vi "XMLPublishNode.vi"(8 "Error In":errorcluster, 9 "parent opcua path":string, 10 "OPC UA server refnum in":refnum<k21>, 11 "DOM node":refnum<k20>) -> (0 "Error Out":errorcluster, 2 "OPC UA server refnum out":refnum<k21>, 3 "DOM node (dup)":refnum<k20>)   [LabVIEW 2014, in "OPCUA XML(dev).lvlib"]
uses:
  OPCUA XML(dev).lvlib
  <resource>/objmgr/DOMUserDefRef.rc
  <vilib>/xml/NI_XML.lvlib
  <vilib>/xml/Close Reference(Node).vi
  <vilib>/OPCUA/NI OPC UA Server.lvlib
  <vilib>/xml/Close Reference(NNMap).vi
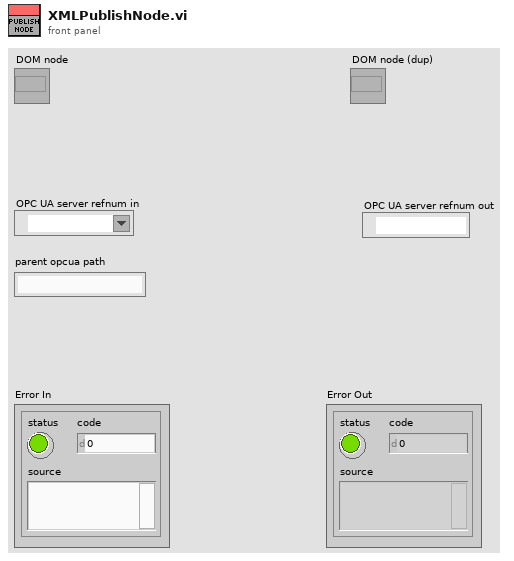
[diagram p1: front panel]
types:
  T1 = cluster{"name":string, "data type":u16, "access level":u16, "description":string}
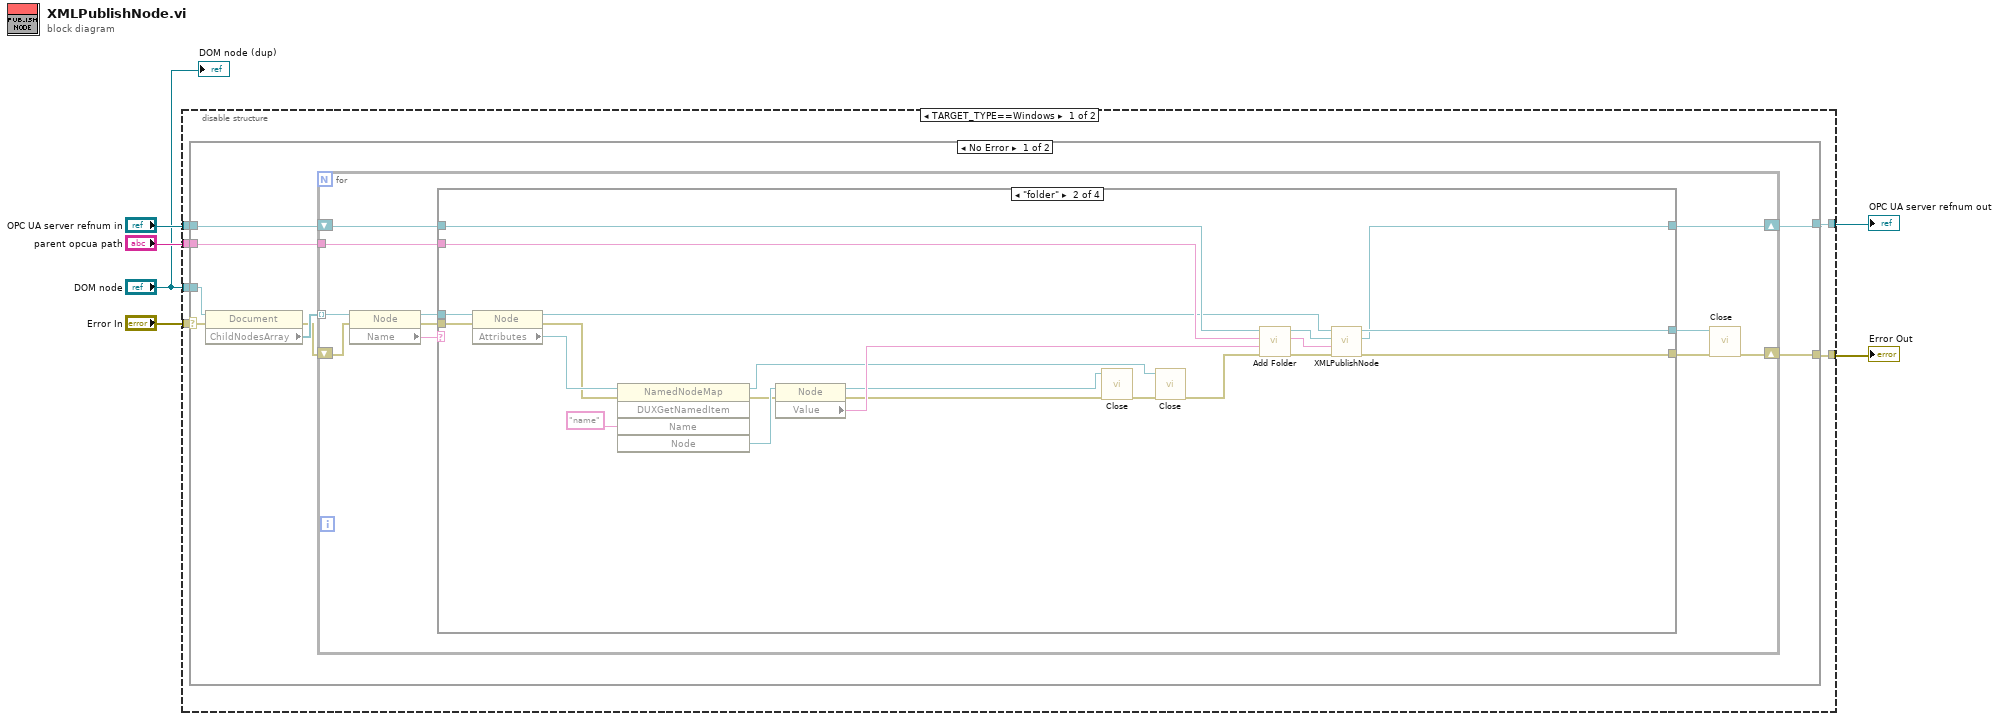
[diagram p0: block diagram]
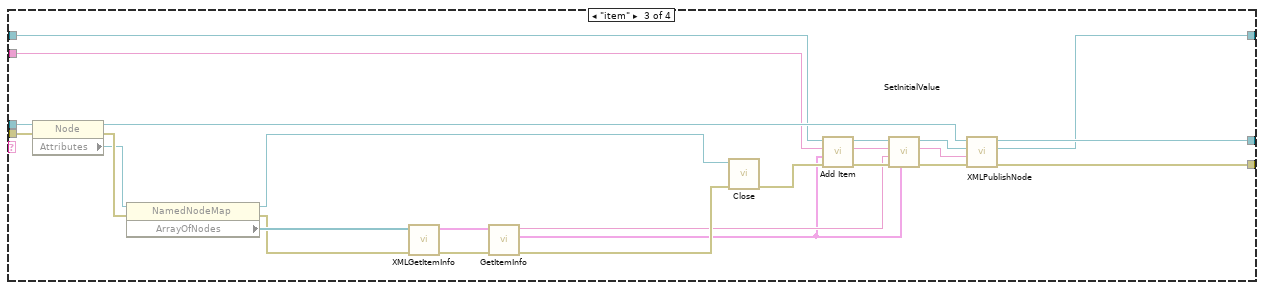
[diagram p3: hidden frame]
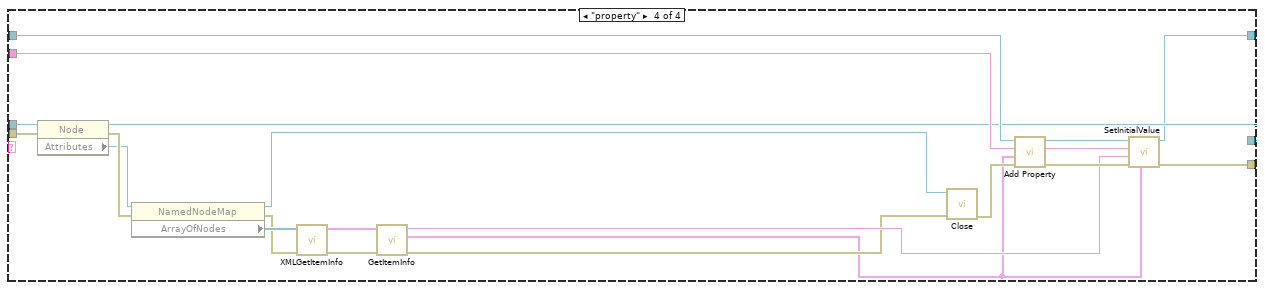
[diagram p4: hidden frame]
diagram:
  n1 = disable-structure shown="TARGET_TYPE==Windows" {
    disable-tunnel: [w12 w105] -> w6
    disable-tunnel: "Error In" -> [w11 w105]
    disable-tunnel: "parent opcua path" -> [w10 _]
    disable-tunnel: "OPC UA server refnum in" -> [w9 w106]
    disable-tunnel: [w8 w106] -> w2
    disable-tunnel: "DOM node" -> [w7 _]
    frame condition #0 {
      n2 = case shown="No Error" w11 {
        selector: w11 -> [w14 w104]
        tunnel: [w18 w104] -> w12
        tunnel: w7 -> [w20 _]
        tunnel: w10 -> [w17 _]
        tunnel: w9 -> [w16 w103]
        tunnel: [w15 w103] -> w8
        frame No Error {
          n3 = property class="Document"(reference=w20, error in=w14) -> (error out=w13:errorcluster, "ChildNodesArray"=w19:refnum<k20>[])  [unwired: 1 out]
          n4 = for {
            tunnel: w19 -> [w31] mode=indexing
            shift-right: [w27] -> w18
            shift-left: w13 -> [w28]
            tunnel: w17 -> [w26]
            shift-right: [w24] -> w15
            shift-left: w16 -> [w25]
            n5 = property class="Node"(reference=w31, error in=w28) -> (reference out=w29:refnum<k20>, error out=w23:errorcluster, "Name"=w30:string)
            n6 = case shown="\"folder\"" w30 {
              tunnel: w29 -> [w33 w56 w81 w97]
              tunnel: w26 -> [_ w52 w77 w101]
              tunnel: w25 -> [w32 w51 w78 w102]
              tunnel: [w32 w45 w76 w91] -> w24
              tunnel: w23 -> [w34 w42 w74 w96]
              tunnel: [w33 w48 w80 w95] -> w22
              tunnel: [w34 w47 w75 w90] -> w21
              frame Default {
              }
              frame "folder" {
                n7 = property class="Node"(reference=w56, error in=w42) -> (reference out=w49:refnum<k20>, error out=w41:errorcluster, "Attributes"=w55:refnum<k20>)
                n8 = invoke class="NamedNodeMap" method="DUXGetNamedItem"(reference=w55, error in=w41, "Name"="name") -> (reference out=w36:refnum<k20>, error out=w40:errorcluster, "Node"=w53:refnum<k20>)  [unwired: 2 in, 2 out]
                n9 = property class="Node"(reference=w53, error in=w40) -> (reference out=w35:refnum<k20>, error out=w39:errorcluster, "Value"=w50:string)
                n10 = call-poly <vilib>:"Close.vi"("error in (no error)"=w39, "node"=w35) -> ("error out"=w38:errorcluster)  [unwired: 7 out]
                n11 = call-poly <vilib>:"Close.vi"("error in (no error)"=w38, "named node map"=w36) -> ("error out"=w37:errorcluster)  [unwired: 7 out]
                n12 = call <vilib>:"Add Folder.vi"("error in (no error)"=w37, "folder name"=w50, "parent folder path"=w52, "OPC UA server refnum in"=w51) -> ("error out"=w43:errorcluster, "folder path"=w44:string, "OPC UA server refnum out"=w46:refnum<k21>)  [unwired: 4 in]
                n13 = call "XMLPublishNode.vi"("Error In"=w43, "parent opcua path"=w44, "OPC UA server refnum in"=w46, "DOM node"=w49) -> ("Error Out"=w47:errorcluster, "OPC UA server refnum out"=w45:refnum<k21>, "DOM node (dup)"=w48:refnum<k20>)  [unwired: 5 in]
              }
              frame "item" {
                n14 = property class="Node"(reference=w81, error in=w74) -> (reference out=w79:refnum<k20>, error out=w73:errorcluster, "Attributes"=w72:refnum<k20>)
                n15 = property class="NamedNodeMap"(reference=w72, error in=w73) -> (reference out=w71:refnum<k20>, error out=w62:errorcluster, "ArrayOfNodes"=w63:refnum<k20>[])
                n16 = call "XMLGetItemInfo.vi"("error in (no error)"=w62, "ArrayOfNodes"=w63) -> ("error out"=w61:errorcluster, "Array"=w60:cluster{"Name":string, "Value":string}[])  [unwired: 8 in]
                n17 = call "GetItemInfo.vi"("error in (no error)"=w61, "Array"=w60) -> ("error out"=w59:errorcluster, "item"=w57:T1, "Value"=w58:string)  [unwired: 7 in]
                n18 = call-poly <vilib>:"Close.vi"("error in (no error)"=w59, "named node map"=w71) -> ("error out"=w70:errorcluster)  [unwired: 7 out]
                n19 = call <vilib>:"Add Item.vi"("error in (no error)"=w70, "item"=w57, "parent folder path"=w77, "OPC UA server refnum in"=w78) -> ("error out"=w67:errorcluster, "item path"=w68:string, "OPC UA server refnum out"=w69:refnum<k21>)  [unwired: 4 in]
                n20 = call "SetInitialValue.vi"("item"=w57, "Error In"=w67, "value string"=w58, "node path"=w68, "OPC UA server refnum in"=w69) -> ("Error Out"=w66:errorcluster, "node path (dup)"=w64:string, "OPC UA server refnum out"=w65:refnum<k21>)  [unwired: 4 in]
                n21 = call "XMLPublishNode.vi"("Error In"=w66, "parent opcua path"=w64, "OPC UA server refnum in"=w65, "DOM node"=w79) -> ("Error Out"=w75:errorcluster, "OPC UA server refnum out"=w76:refnum<k21>, "DOM node (dup)"=w80:refnum<k20>)  [unwired: 5 in]
              }
              frame "property" {
                n22 = property class="Node"(reference=w97, error in=w96) -> (reference out=w95:refnum<k20>, error out=w100:errorcluster, "Attributes"=w99:refnum<k20>)
                n23 = property class="NamedNodeMap"(reference=w99, error in=w100) -> (reference out=w98:refnum<k20>, error out=w85:errorcluster, "ArrayOfNodes"=w86:refnum<k20>[])
                n24 = call "XMLGetItemInfo.vi"("error in (no error)"=w85, "ArrayOfNodes"=w86) -> ("error out"=w88:errorcluster, "Array"=w87:cluster{"Name":string, "Value":string}[])  [unwired: 8 in]
                n25 = call "GetItemInfo.vi"("error in (no error)"=w88, "Array"=w87) -> ("error out"=w83:errorcluster, "item"=w82:T1, "Value"=w84:string)  [unwired: 7 in]
                n26 = call-poly <vilib>:"Close.vi"("error in (no error)"=w83, "named node map"=w98) -> ("error out"=w94:errorcluster)  [unwired: 7 out]
                n27 = call <vilib>:"Add Property.vi"("error in (no error)"=w94, "property"=w82, "item path"=w101, "OPC UA server refnum in"=w102) -> ("error out"=w92:errorcluster, "property path"=w89:string, "OPC UA server refnum out"=w93:refnum<k21>)  [unwired: 4 in]
                n28 = call "SetInitialValue.vi"("item"=w82, "Error In"=w92, "value string"=w84, "node path"=w89, "OPC UA server refnum in"=w93) -> ("Error Out"=w90:errorcluster, "OPC UA server refnum out"=w91:refnum<k21>)  [unwired: 4 in, 1 out]
              }
            }
            n29 = call-poly <vilib>:"Close.vi"("error in (no error)"=w21, "node"=w22) -> ("error out"=w27:errorcluster)  [unwired: 7 out]
          }
        }
        frame Error {
        }
      }
    }
    frame condition #1 (active) {
    }
  }
  "Error Out" <- w6
  "OPC UA server refnum out" <- w2
  "DOM node (dup)" <- "DOM node"
